vi "Test Comm MODBUS.vi"(2 "Adresse rég":u8 caption="Adresse régulateur", 3 "Port COM run 1 REG":refnum<visa-resource-name> caption="Port RS232") -> (0 "error out":errorcluster)   [LabVIEW 2022 SP3]
uses:
  Variables globales/Variables glob EUROTHERM.vi
panel:
  out "Nom rég":string caption="Nom régulateur"
  # "test COM"
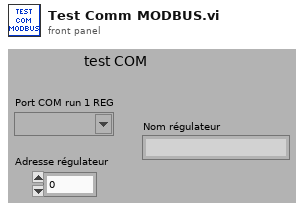
[diagram p1: front panel]
types:
  T1 = typedef "Semaphore RefNum" = refnum<k1>
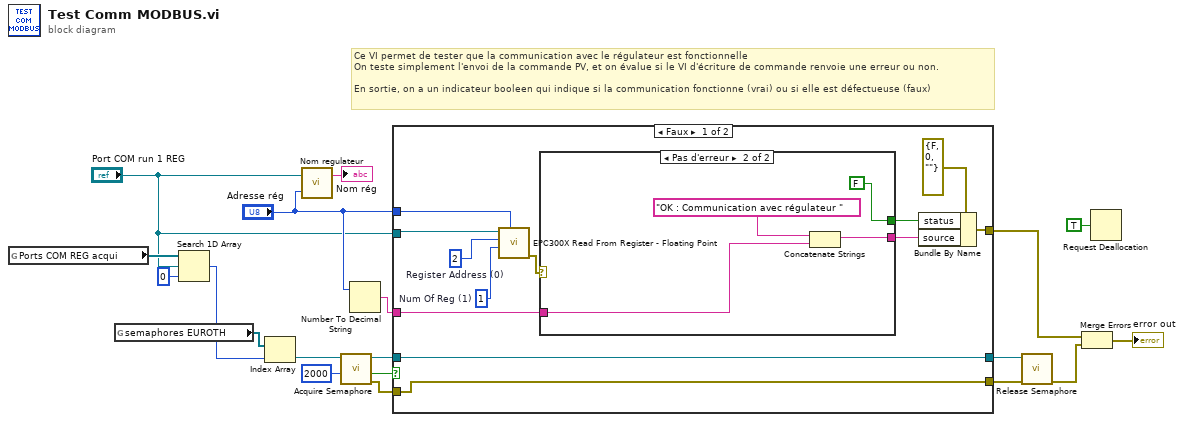
[diagram p0: block diagram]
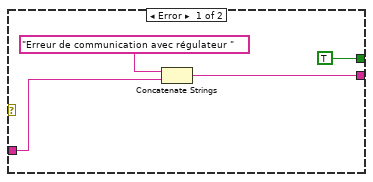
[diagram p2: hidden frame]
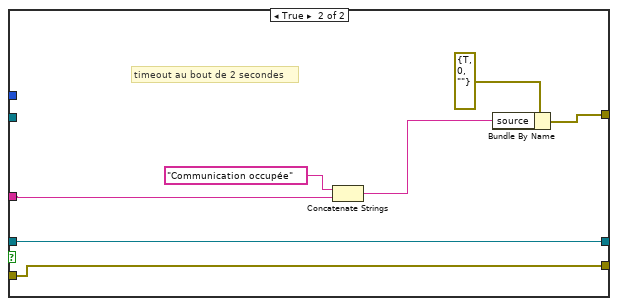
[diagram p3: hidden frame]
diagram:
  # "Ce VI permet de tester que la communication avec le régulateur est fonctionnelle\nOn teste simplement l'envoi de la commande PV, et on évalue si le VI d'écriture de commande renvoie une erreur ou non.\n\nEn sortie, on a un indicateur booleen qui indique si la communication fonctionne (vrai) ou si elle est défectueuse (faux)"
  n1 = global read "Variables glob EUROTHERM.vi" "Ports COM REG acqui"() -> (w4:refnum<visa-resource-name>[])
  n2 = global read "Variables glob EUROTHERM.vi" "semaphores EUROTH"() -> (w8:T1[])
  n3 = Search 1D Array(1D array=w4, element="Port COM run 1 REG", start index (0)=0 ("indice de départ (0)")) -> (index of element=w1:i32)
  n4 = Index Array(array=w8, index=w1) -> (element=w7:T1)
  n5 = call "Nom regulateur.vi"("Adresse régulateur"="Adresse rég", "Port COM run 1 REG"="Port COM run 1 REG") -> ("Nom régulateur"=→"Nom rég":string)  [unwired: 1 in]
  n6 = call <vilib>:"Acquire Semaphore.vi"("ms timeout (-1)"=2000, "semaphore"=w7) -> ("error out"=w16:errorcluster, "timed out"=w17:bool, "semaphore out"=w15:T1)  [unwired: 3 in]
  n7 = Number To Decimal String(number="Adresse rég") -> (decimal integer string=w12:string)  [unwired: 1 in]
  n8 = case shown="Faux" w17 {
    tunnel: w16 -> [w30 w43]
    tunnel: w15 -> [w31 w44]
    tunnel: [w31 w44] -> w14
    tunnel: [w30 w43] -> w13
    tunnel: "Adresse rég" -> [w20 _]
    tunnel: w12 -> [w29 w45]
    tunnel: [w26 w40] -> w10
    tunnel: "Port COM run 1 REG" -> [w21 _]
    frame False {
      w23 = u16 2  # Register Address (0)
      w24 = u16 1  # Num Of Reg (1)
      n9 = call "EPC300X Read From Register - Floating Point.vi"("Unit Address (1)"=w20, "Num Of Reg (1)"=w24, "Register Address (0)"=w23, "VISA session"=w21) -> ("error out"=w22:errorcluster)  [unwired: 2 in, 5 out]
      n10 = case shown="Pas d'erreur" w22 {
        tunnel: w29 -> [w35 w39]
        tunnel: [w33 w37] -> w27
        tunnel: [TRUE FALSE] -> w25
        frame Error {
          n11 = Concatenate Strings("Erreur de communication avec régulateur ", w35) -> (w33:string)
        }
        frame No Error {
          n12 = Concatenate Strings("OK : Communication avec régulateur ", w39) -> (w37:string)
        }
      }
      n13 = Bundle By Name(cluster=errorcluster {"status"=FALSE, "code"=0, "source"=""} ("error out"), "status"=w25, "source"=w27) -> (w26:errorcluster)
    }
    frame True {
      # "timeout au bout de 2 secondes"
      n14 = Concatenate Strings("Communication occupée", w45) -> (w41:string)
      n15 = Bundle By Name(cluster=errorcluster {"status"=TRUE, "code"=0, "source"=""} ("error out"), "source"=w41) -> (w40:errorcluster)
    }
  }
  n16 = call <vilib>:"Release Semaphore.vi"("error in (no error)"=w13, "semaphore"=w14) -> ("error out"=w11:errorcluster)  [unwired: 4 in, 1 out]
  n17 = Merge Errors(w10, w11) -> (→"error out":errorcluster)
  n18 = Request Deallocation(TRUE ("flag")) -> ()
